vi "DSS-Tests-flatten_common_format.vi"(11 "Common Format":T1) -> (3 "flat":dbl[](array[numeric]))   [LabVIEW 2020, in "DSS-Tests.lvlib"]
doc: "Flattens a Common Format cluster into one 1D DBL array: for each of its nine arrays in cluster order, the length followed by the elements."
uses:
  DSS-Tests.lvlib
  Reflector/RFH-common_data_format.ctl
  Reflector/RFH-Reflection_File_Handler.lvlib
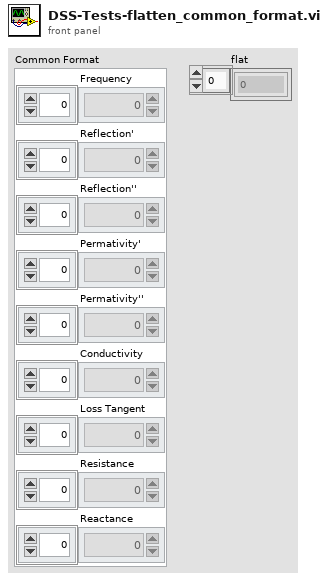
[diagram p1: front panel]
types:
  T1 = typedef "RFH-Reflection_File_Handler.lvlib/RFH-common_data_format.ctl" = cluster{"Frequency":dbl[], "Reflection'":dbl[], "Reflection''":dbl[], "Permativity'":dbl[], "Permativity''":dbl[], "Conductivity":dbl[], "Loss Tangent":dbl[], "Resistance":dbl[], "Reactance":dbl[]}
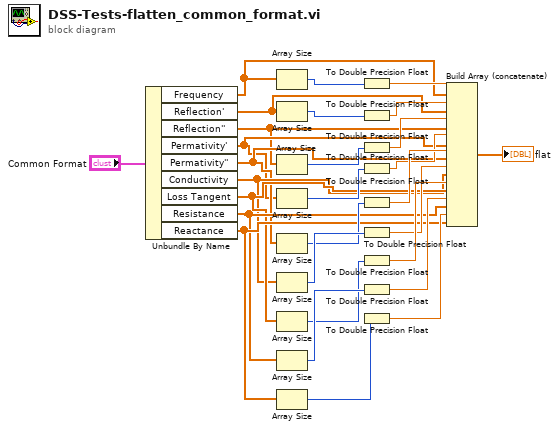
[diagram p0: block diagram]
diagram:
  n1 = Unbundle By Name("Common Format") -> ("Frequency"=w2:dbl[], "Reflection'"=w3:dbl[], "Reflection''"=w4:dbl[], "Permativity'"=w5:dbl[], "Permativity''"=w6:dbl[], "Conductivity"=w7:dbl[], "Loss Tangent"=w8:dbl[], "Resistance"=w9:dbl[], "Reactance"=w10:dbl[])
  n2 = Array Size(array=w2) -> (size(s)=w11:i32)
  n3 = Array Size(array=w3) -> (size(s)=w13:i32)
  n4 = Array Size(array=w4) -> (size(s)=w15:i32)
  n5 = Array Size(array=w5) -> (size(s)=w17:i32)
  n6 = Array Size(array=w6) -> (size(s)=w19:i32)
  n7 = Array Size(array=w7) -> (size(s)=w21:i32)
  n8 = Array Size(array=w8) -> (size(s)=w23:i32)
  n9 = Array Size(array=w9) -> (size(s)=w25:i32)
  n10 = Array Size(array=w10) -> (size(s)=w27:i32)
  n11 = To Double Precision Float(number=w11) -> (double precision float=w12:dbl)
  n12 = To Double Precision Float(number=w13) -> (double precision float=w14:dbl)
  n13 = To Double Precision Float(number=w15) -> (double precision float=w16:dbl)
  n14 = To Double Precision Float(number=w17) -> (double precision float=w18:dbl)
  n15 = To Double Precision Float(number=w19) -> (double precision float=w20:dbl)
  n16 = To Double Precision Float(number=w21) -> (double precision float=w22:dbl)
  n17 = To Double Precision Float(number=w23) -> (double precision float=w24:dbl)
  n18 = To Double Precision Float(number=w25) -> (double precision float=w26:dbl)
  n19 = To Double Precision Float(number=w27) -> (double precision float=w28:dbl)
  n20 = Build Array (concatenate)(w12, w2, w14, w3, w16, w4, w18, w5, w20, w6, w22, w7, w24, w8, w26, w9, w28, w10) -> (→"flat":dbl[])
